vi "FuncVI-Imag.vi"(5 "InstanceRef":T2, 9 "arg list":T1[](array[typedef]) {"num" format="%.2f"}) -> (0 "error out":bool, 3 "result":T1 {"num" format="%.2f"})   [LabVIEW 2021]
doc: "::: CalcExpress Toolkit :::\nCopyright (c) 2000-2026 Konstantin Shifershteyn. All rights reserved."
uses:
  cetypes.llb/CalcExpress Function Argument Info.ctl
  cetypes.llb/CalcExpress Instance RefNum.ctl
panel:
  in  "max arg num":i32=1
  in  "min arg num":i32=1
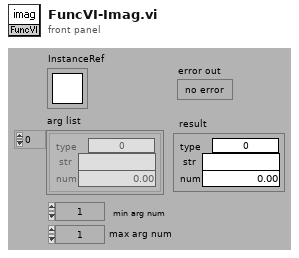
[diagram p1: front panel]
types:
  T1 = typedef "CalcExpress Function Argument Info.ctl" = cluster{"type":u32, "str":string, "num":dbl}
  T2 = typedef "CalcExpress Instance RefNum.ctl" = refnum<k1>
  T3 = enum16{"DBL scalar", "CDB scalar", "DBL array", "CDB array", "ERROR"}
  T4 = typedef "CalcExpress Data Type.ctl" = enum32{"String", "DBL Number", "identifier", "1D Array of DBL", "2D Array of DBL", "CDB Number", "1D Array of CDB", "2D Array of CDB", "1D Array of String", "2D Array of String", "Unknown data type"}
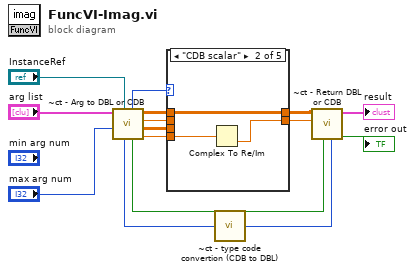
[diagram p0: block diagram]
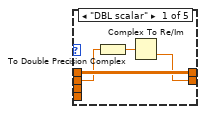
[diagram p2: hidden frame]
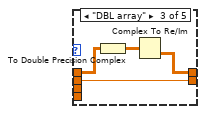
[diagram p3: hidden frame]
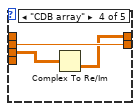
[diagram p4: hidden frame]
diagram:
  n1 = call "~ct - Arg to DBL or CDB.vi"("InstanceRef"="InstanceRef", "max args"="max arg num", "args list"="arg list") -> ("CDB"=w9:cdb, "2D CDB"=w10:cdb[][], "DBL"=w8:dbl, "2D DBL"=w7:dbl[][], "error out"=w11:bool, "category"=w4:T3, "arg type"=w3:T4)  [unwired: 2 in]
  n2 = case shown="\"CDB scalar\"" w4 {
    tunnel: w10 -> [_ _ _ w28 _]
    tunnel: w9 -> [_ w21 _ _ _]
    tunnel: w8 -> [w18 _ w26 w29 w30]
    tunnel: w7 -> [w19 w22 w25 _ w31]
    tunnel: [w19 w22 w23 w27 w31] -> w6
    tunnel: [w16 w20 w26 w29 w30] -> w5
    frame "DBL scalar" {
      n3 = To Double Precision Complex(1:w18) -> (0:w17:cdb)
      n4 = Complex To Re/Im(x + iy=w17) -> (y=w16:dbl)  [unwired: 1 out]
    }
    frame "CDB scalar" {
      n5 = Complex To Re/Im(x + iy=w21) -> (y=w20:dbl)  [unwired: 1 out]
    }
    frame "DBL array" {
      n6 = To Double Precision Complex(1:w25) -> (0:w24:cdb[][])
      n7 = Complex To Re/Im(x + iy=w24) -> (y=w23:dbl[][])  [unwired: 1 out]
    }
    frame "CDB array" {
      n8 = Complex To Re/Im(x + iy=w28) -> (y=w27:dbl[][])  [unwired: 1 out]
    }
    frame "ERROR" {
    }
  }
  n9 = call "~ct - type code convertion (CDB to DBL).vi"("type"=w3) -> ("type out"=w2:T4)  [unwired: 4 in]
  n10 = call "~ct - Return DBL or CDB.vi"("type"=w2, "error in"=w11, "DBL"=w5, "2D DBL"=w6) -> ("error out"=→"error out":bool, "result"=→"result":T1)  [unwired: 6 in]
